vi "Discover XNET CAN.vi"(8 "error in (no error)":errorcluster) -> (0 "error out":errorcluster, 3 "XNET Devices":T1[](array[typedef]))   [LabVIEW 2021, in "XNET CAN RW.lvclass"]
uses:
  XNET CAN RW.lvclass
  XNET CAN RW.lvclass/XNET CAN RW.ctl
  <resource>/objmgr/xnet.rc
  <vilib>/regexp/Match Regular Expression.xnode
  typedef/XNET Devices.ctl
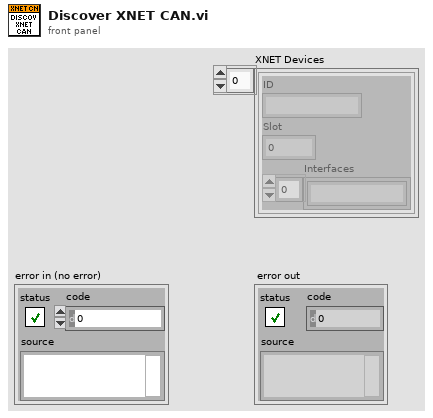
[diagram p1: front panel]
types:
  T1 = typedef "XNET CAN RW.lvclass/XNET Devices.ctl" = cluster{"ID":string, "Slot":u32, "Interfaces":string[]}
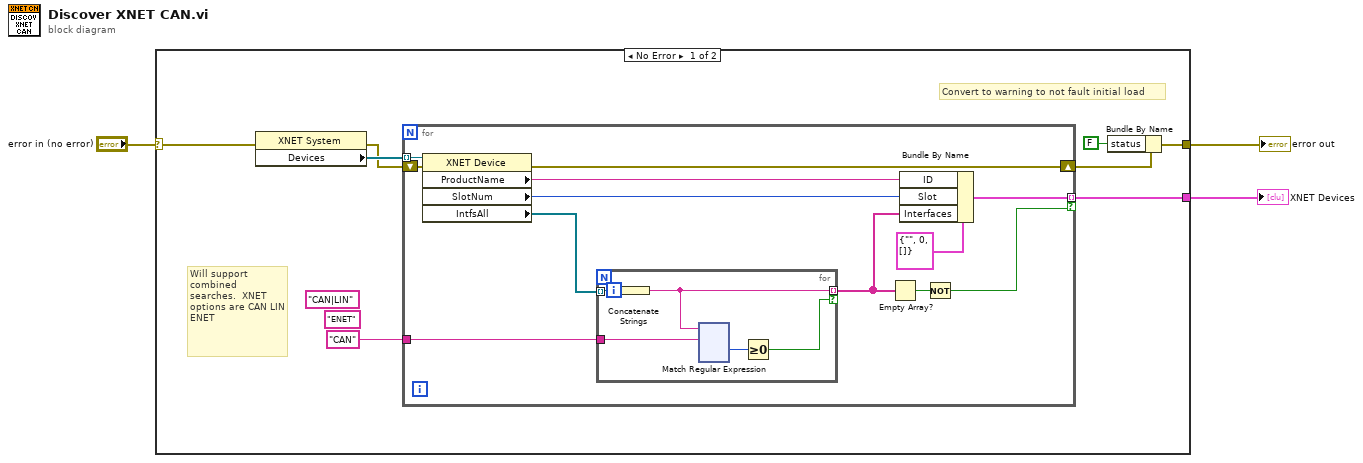
[diagram p0: block diagram]
diagram:
  n1 = case shown="No Error" "error in (no error)" {
    selector: "error in (no error)" -> [w7 w146]
    tunnel: [w4 w146] -> w3
    tunnel: [w8 _] -> w2
    frame No Error {
      (unwired) "ENET" ("regular expression")
      (unwired) "CAN|LIN" ("regular expression")
      # "Convert to warning to not fault initial load"
      # "Will support combined searches.  XNET options are CAN LIN ENET"
      n2 = property class="XNET System"(error in=w7) -> (error out=w10:errorcluster, "Devices"=w11:refnum<k21>[])  [unwired: 1 in, 1 out]
      n3 = for {
        tunnel: w11 -> [w23] mode=indexing
        tunnel: [w21] -> w8 mode=indexing if=w12
        shift-right: [w19] -> w5
        shift-left: w10 -> [w20]
        tunnel: "CAN" ("regular expression") -> [w15]
        n4 = property class="XNET Device"(reference=w23, error in=w20) -> (error out=w19:errorcluster, "ProductName"=w18:string, "SlotNum"=w17:u32, "IntfsAll"=w22:refnum<k21>[])  [unwired: 1 out]
        n5 = for {
          tunnel: w22 -> [w28] mode=indexing
          tunnel: [w27] -> w14 mode=indexing if=w24
          tunnel: w15 -> [w26]
          n6 = Concatenate Strings(w28) -> (w27:string)
          n7 = xnode "Match Regular Expression"("input string"=w27, "regular expression"=w26) -> ("offset past match"=w25:i32)  [unwired: 4 in, 4 out]
          n8 = Greater Or Equal To 0?(x=w25) -> (x >= 0?=w24:bool)
        }
        n9 = Empty Array?(array=w14) -> (empty?=w13:bool)
        n10 = Bundle By Name(cluster=T1 {"ID"="", "Slot"=0, "Interfaces"=[]} ("UDP_Writer_XNETInfo_Board"), "ID"=w18, "Slot"=w17, "Interfaces"=w14) -> (w21:T1)
        n11 = Not(x=w13) -> (.not. x?=w12:bool)
      }
      n12 = Bundle By Name(cluster=w5, "status"=FALSE) -> (w4:errorcluster)
    }
    frame Error {
    }
  }
  "error out" <- w3
  "XNET Devices" <- w2
